vi "thermal_optical_camera_5.vi"() -> ()   [LabVIEW 2025]
panel:
  in  "Focus":dbl(slide) scale=0.0..100.0
  out "Currently written frame":string
  in  "Thermal output folder":path
  in  "thermal capture interval (s)":dbl
  in  "Flag Button":bool
  in  "Stop & Save":bool
  in  "Stop Preview":bool
  in  "Record":bool
  # "(1) Run VI"
  # "(2) After thermal camera calibration message (in terminal), press START"
  # "(3) Stop & Save"
  # "(Enter \"28\")"
  # "Thermal Record"
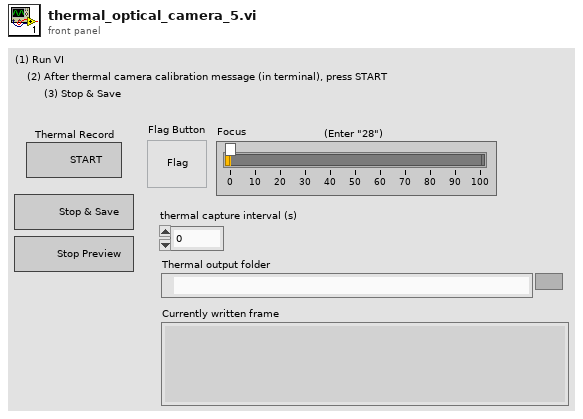
[diagram p1: front panel]
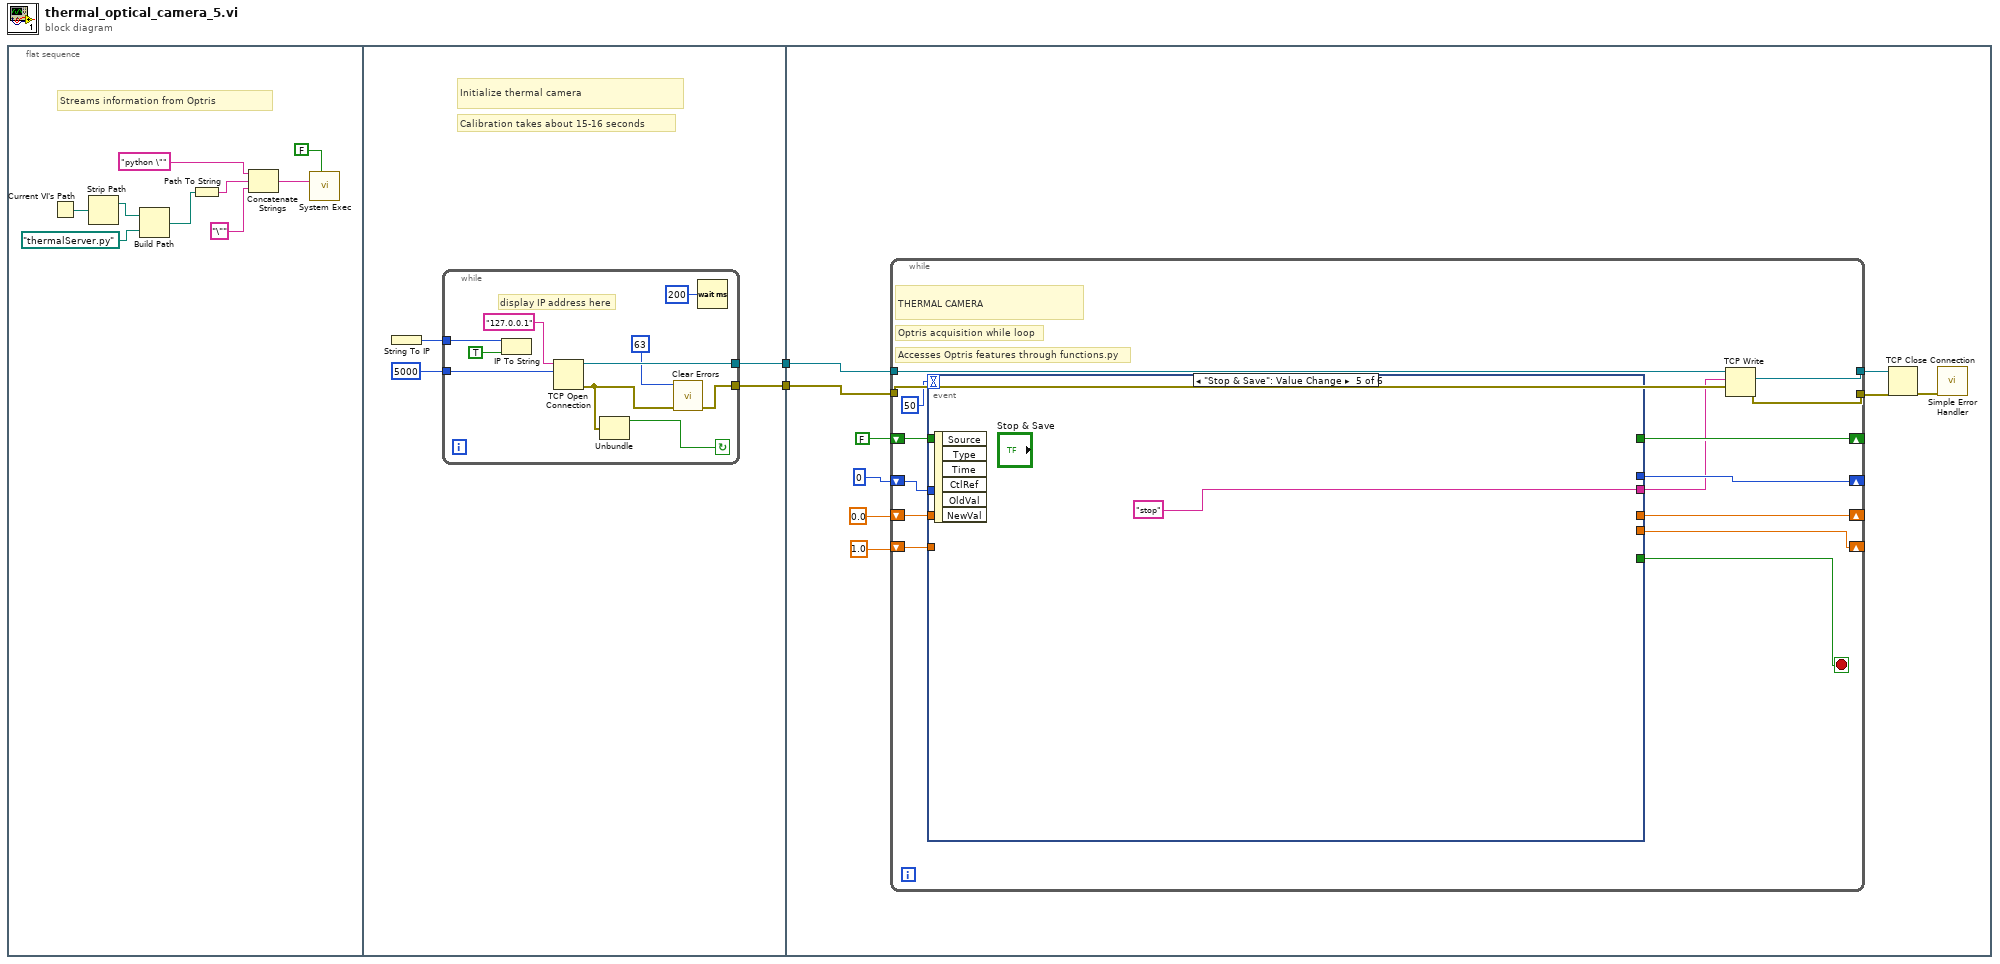
[diagram p0: block diagram]
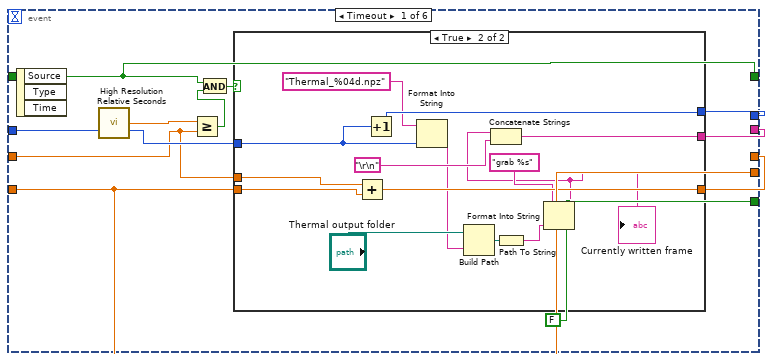
[diagram p2: hidden frame]
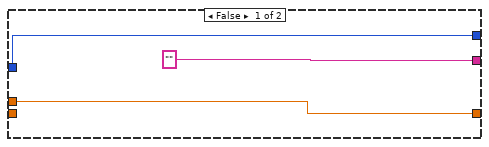
[diagram p3: hidden frame]
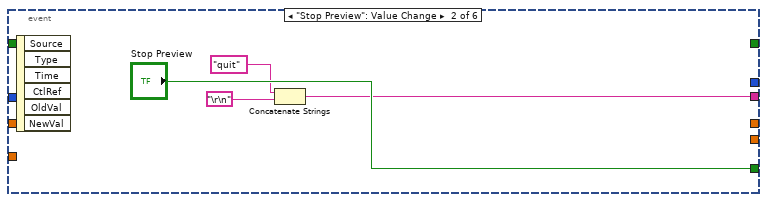
[diagram p4: hidden frame]
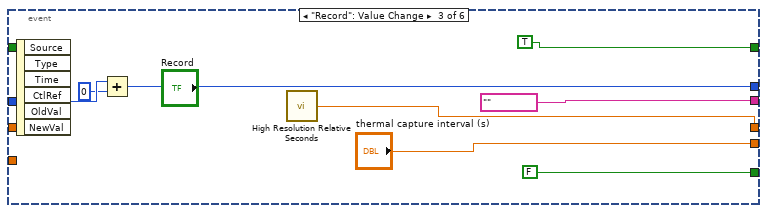
[diagram p5: hidden frame]
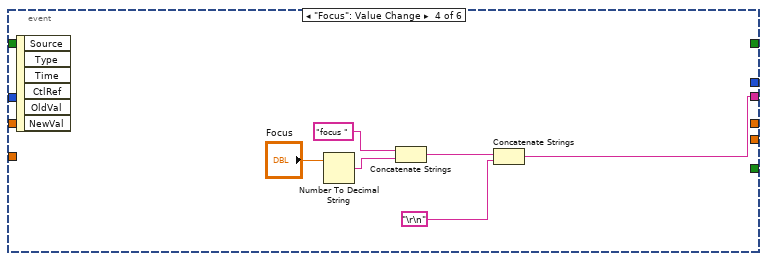
[diagram p6: hidden frame]
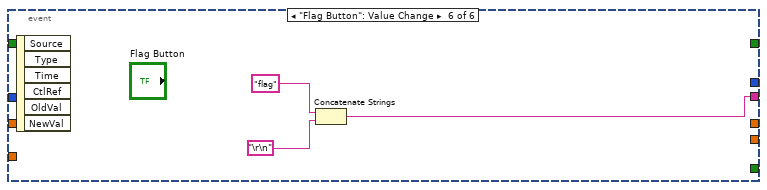
[diagram p7: hidden frame]
diagram:
  n1 = flat-sequence {
    tunnel: [w13] -> w2
    tunnel: [w12] -> w1
    tunnel: w1 -> [w31]
    tunnel: w2 -> [w30]
    frame #0 {
      # "Streams information from Optris"
      n2 = Current VI's Path() -> (path=w6:path)
      n3 = Strip Path(path=w6) -> (stripped path=w7:path)  [unwired: 1 out]
      n4 = Build Path(base path=w7, name or relative path=path "thermalServer.py") -> (appended path=w4:path)
      n5 = Path To String(path=w4) -> (string=w10:string)
      n6 = Concatenate Strings("python \"" ("string"), w10, "\"" ("string")) -> (w9:string)
      n7 = call <vilib>:"System Exec.vi"("wait until completion? (T)"=FALSE, "command line"=w9) -> ()  [unwired: 6 in, 4 out]
    }
    frame #1 {
      # "Initialize thermal camera"
      # "Calibration takes about 15-16 seconds"
      n8 = String To IP() -> (0:w15:u32)  [unwired: 1 in]
      n9 = while {
        tunnel: [w20] -> w13
        tunnel: [w25] -> w12
        tunnel: w15 -> [w24]
        tunnel: u16 5000 ("remote port or service name") -> [w22]
        stop <- w17 continue-if-true
        # "display IP address here"
        n10 = IP To String(1:TRUE ("dot notation? (F)"), 2:w24) -> ()  [unwired: 1 out]
        n11 = TCP Open Connection(address="127.0.0.1", remote port or service name=w22) -> (connection ID=w25:refnum<k5>, error out=w21:errorcluster)  [unwired: 3 in]
        n12 = Unbundle(w21) -> ("status"=w17:bool)  [unwired: 2 out]
        n13 = call <vilib>:"Clear Errors.vi"("error in (no error)"=w21, "specific error code to clear (0: all)"=63) -> ("error out"=w20:errorcluster)  [unwired: 4 in, 1 out]
        n14 = Wait (ms)(milliseconds to wait=u32 200) -> ()  [unwired: 1 out]
      }
    }
    frame #2 {
      n15 = while {
        tunnel: [w49] -> w32
        tunnel: [w48] -> w33
        tunnel: w31 -> [w46]
        tunnel: w30 -> [w45]
        shift-right: [w43] -> _
        shift-left: u32 0 -> [w44]
        shift-right: [w42] -> _
        shift-left: 0.0 -> [w38]
        shift-right: [w39] -> _
        shift-left: 1.0 -> [w36]
        shift-right: [w40] -> _
        shift-left: FALSE -> [w37]
        stop <- w47 stop-if-true
        # "THERMAL CAMERA"
        # "Optris acquisition while loop"
        # "Accesses Optris features through functions.py"
        n16 = event shown="[4] \"Stop & Save\": Value Change" {
          selector: _ -> [_ _ _ _ _ _]
          dyn-events: _ -> [_ _ _ _ _ _]
          timeout: 50 -> [_ _ _ _ _ _]
          tunnel: [w56 w78 "" w90 "stop" w99] -> w35
          tunnel: [FALSE "Stop Preview" FALSE _ _ _] -> w47
          tunnel: w44 -> [w57 _ w89 _ _ _]
          tunnel: [w55 _ w87 _ _ _] -> w43
          tunnel: [w53 _ w86 _ _ _] -> w42
          tunnel: [w51 _ TRUE _ _ _] -> w40
          tunnel: [w52 _ "thermal capture interval (s)" _ _ _] -> w39
          tunnel: w38 -> [w54 _ _ _ _ _]
          tunnel: w37 -> [w51 _ _ _ _ _]
          tunnel: w36 -> [w52 _ _ _ _ _]
          event Timeout {
            n17 = event-data() -> ()  [unwired: 1 in, 3 out]
            n18 = call <vilib>:"High Resolution Relative Seconds.vi"() -> ("relative seconds"=w60:dbl)
            n19 = Greater Or Equal?(x=w60, y=w54) -> (x >= y?=w59:bool)
            n20 = And(x=w51, y=w59) -> (x .and. y?=w58:bool)
            n21 = case shown="True" w58 {
              tunnel: w57 -> [w62 w75]
              tunnel: ["" w76] -> w56
              tunnel: [w62 w74] -> w55
              tunnel: w54 -> [w61 w73]
              tunnel: w52 -> [_ w72]
              tunnel: [w61 w71] -> w53
              frame False {
              }
              frame True {
                n22 = Add(x=w73, y=w72) -> (x+y=w71:dbl)
                n23 = Increment(x=w75) -> (x+1=w74:u32)
                n24 = Format Into String(format string="Thermal_%04d.npz", w75) -> (resulting string=w66:string)  [unwired: 2 in, 1 out]
                n25 = Build Path(base path="Thermal output folder", name or relative path=w66) -> (appended path=w68:path)
                n26 = Path To String(path=w68) -> (string=w65:string)
                n27 = Format Into String(format string="grab %s", w65) -> (resulting string=w64:string)  [unwired: 2 in, 1 out]
                "Currently written frame" <- w64
                n28 = Concatenate Strings(w64, "\r\n") -> (w76:string)
              }
            }
          }
          event "Stop Preview": Value Change {
            n29 = event-data() -> ()  [unwired: 1 in, 6 out]
            n30 = Concatenate Strings("quit", "\r\n") -> (w78:string)
          }
          event "Record": Value Change {
            n31 = event-data() -> ()  [unwired: 1 in, 6 out]
            n32 = Add(x=w89, y=u32 0) -> (x+y=w87:u32)
            n33 = call <vilib>:"High Resolution Relative Seconds.vi"() -> ("relative seconds"=w86:dbl)
          }
          event "Focus": Value Change {
            n34 = event-data() -> ()  [unwired: 1 in, 6 out]
            n35 = Number To Decimal String(number="Focus") -> (decimal integer string=w95:string)  [unwired: 1 in]
            n36 = Concatenate Strings("focus ", w95) -> (w92:string)
            n37 = Concatenate Strings(w92, "\r\n") -> (w90:string)
          }
          event "Stop & Save": Value Change {
            n38 = event-data() -> ()  [unwired: 1 in, 6 out]
          }
          event "Flag Button": Value Change {
            n39 = event-data() -> ()  [unwired: 1 in, 6 out]
            n40 = Concatenate Strings("flag", "\r\n") -> (w99:string)
          }
        }
        n41 = TCP Write(connection ID=w46, data in=w35, error in (no error)=w45) -> (connection ID out=w48:refnum<k5>, error out=w49:errorcluster)  [unwired: 1 in, 1 out]
      }
      n42 = TCP Close Connection(connection ID=w33, error in (no error)=w32) -> (error out=w34:errorcluster)  [unwired: 1 in, 1 out]
      n43 = call <vilib>:"Simple Error Handler.vi"("error in (no error)"=w34) -> ()  [unwired: 4 in, 5 out]
    }
  }
